vi "Check for Ini files and create.vi"(11 "User VI Ref":refnum<vi>) -> (0 "error out":errorcluster, 3 "User VI Ref Out":refnum<vi>)   [LabVIEW 2023]
doc: "Check if class, property, and method files exist for current version of LabVIEW, and if not, create them. \n\nRead files into the property array action engine so data is ready for use.\n\nThis is launched asynchronously when plugin runs, so it should only happen once per LabVIEW version."
panel:
  out "(Re)Building helper files":bool
  # "Checks for BundleMagic ini files, and if they don't exist, creates them"
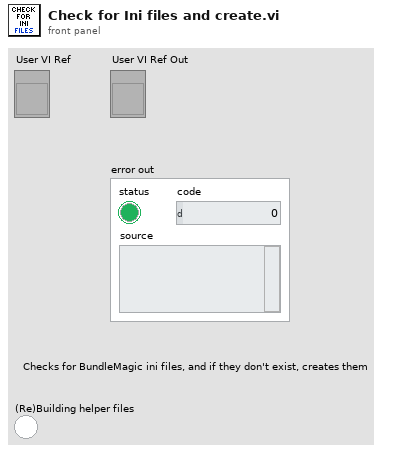
[diagram p1: front panel]
types:
  T1 = cluster{"All files found":bool, "New LV Version (no files found for current version)":bool, "First Run (no files found)":bool}
  T2 = cluster{"First Run":bool, "New LV Version":bool, "Scripting On":bool, "Private On":bool}
  T3 = cluster{"Class Info":cluster{"Unique ID string":string, "Parent ID string":string, "Class Name (unlocalized)":string, "Class Name (localized)":string}, "Method Info":cluster{"Unique ID string":string, "Data name":string, "Short name (localized)":string, "Long name (localized)":string}, "Method Flags":cluster{"IsDeprecated":bool, "IsPrivate":bool, "IsScripting":bool, "IsNotInRun-Time":bool}, "Divider":bool}[]
  T4 = cluster{"Class":cluster{"Unique ID string":string, "Parent ID string":string, "Class Name (unlocalized)":string, "Class Name (localized)":string}, "Property":cluster{"Unique ID string":string, "Data name":string, "Short name (localized)":string, "Long name (localized)":string}, "Flags":cluster{"CanRead":bool, "CanWrite":bool, "IsDeprecated":bool, "IsPrivate":bool, "IsScripting":bool, "IsNotInRun-Time":bool, "Is Reference":bool, "Class Name":string}, "Divider":bool, "Is Write":bool, "Unwired":bool}[]
  T5 = cluster{"Class Info":cluster{"Unique ID string":string, "Parent ID string":string, "Class Name (unlocalized)":string, "Class Name (localized)":string}, "Class Heirarchy":string, "Class Type":enum16{"Unknown", "Base", "Scripting", "Private", "Deprecated", "None", "Divider"}, "Indent":u32}[]
  T6 = cluster{"Done":refnum<user-event>, "Msg 1":refnum<user-event>, "Msg 2":refnum<user-event>, "Prog Max":refnum<user-event>, "Prog Ct":refnum<user-event>}
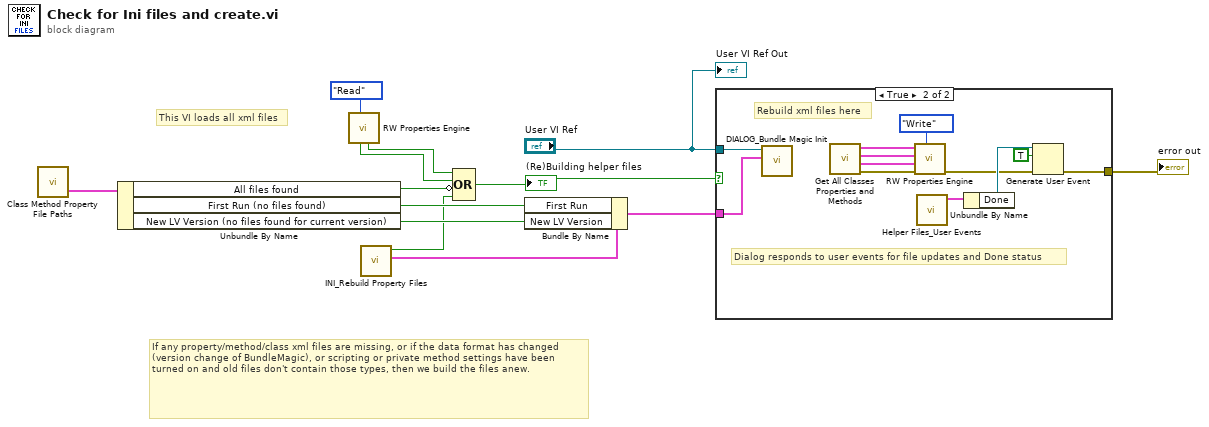
[diagram p0: block diagram]
diagram:
  # "If any property/method/class xml files are missing, or if the data format has changed (version change of BundleMagic), or scripting or private method settings have been turned on and old files don't contain those types, then we build the files anew."
  # "This VI loads all xml files"
  n1 = call "Class Method Property File Paths.vi"() -> ("Files Found Cluster"=w10:T1)  [unwired: 7 in, 4 out]
  n2 = Unbundle By Name(w10) -> ("All files found"=w9:bool, "First Run (no files found)"=w7:bool, "New LV Version (no files found for current version)"=w4:bool)
  n3 = call "RW Properties Engine.vi"("File Action [Read]"=enum16{"Read", "Write"}."Read") -> ("data missing?"=w11:bool, "Data format changed"=w12:bool)  [unwired: 5 in, 4 out]
  n4 = call "INI_Rebuild Property Files.vi"() -> ("Why are we here?"=w8:T2, "Rebuild Property Files"=w3:bool)  [unwired: 10 in]
  n5 = Compound Arithmetic op=OR(w11, w12, invert w9, w3) -> (w5:bool)
  "(Re)Building helper files" <- w5
  n6 = Bundle By Name(cluster=w8, "First Run"=w7, "New LV Version"=w4) -> (w6:T2)
  n7 = case shown="True" w5 {
    tunnel: w6 -> [_ w15]
    tunnel: [_ w16] -> w2
    tunnel: "User VI Ref" -> [_ w14]
    frame False {
    }
    frame True {
      # "Dialog responds to user events for file updates and Done status"
      # "Rebuild xml files here"
      n8 = call "DIALOG_Bundle Magic Init.vi"("Why are we here?"=w15, "Stationary VI Ref"=w14) -> ()  [unwired: 10 in]
      n9 = call "Get All Classes Properties and Methods.vi"() -> ("error out"=w21:errorcluster, "Methods[]"=w22:T3, "Properties[]"=w23:T4, "Classes[]"=w24:T5)  [unwired: 8 in]
      n10 = call "RW Properties Engine.vi"("File Action [Read]"=enum16{"Read", "Write"}."Write", "error in"=w21, "Methods[]"=w22, "Properties[]"=w23, "Classes[]"=w24) -> ("error out"=w17:errorcluster)  [unwired: 1 in, 5 out]
      n11 = call "Helper Files_User Events.vi"() -> ("Init Dialog UEs"=w20:T6)  [unwired: 11 in]
      n12 = Unbundle By Name(w20) -> ("Done"=w19:refnum<user-event>)
      n13 = Generate User Event(user event=w19, event data cluster=TRUE ("event data"), error in=w17) -> (error out=w16:errorcluster)  [unwired: 1 in, 1 out]
    }
  }
  "error out" <- w2
  "User VI Ref Out" <- "User VI Ref"
